vi "K_S30 CalculateCRC16.vi"(7 "msg without CRC":u8[](array[numeric])) -> (0 "CRC16":u16, 1 "CRC Lo":u8, 2 "CRC Hi":u8, 3 "msg and CRC":u8[](array[numeric]))   [LabVIEW 2022 SP3]
panel:
  # "Calculate CRC-16 checksum and append it to the message\nV1.0, b.v."
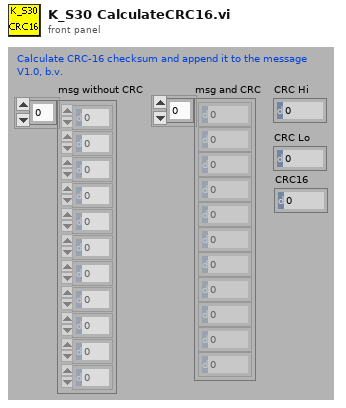
[diagram p1: front panel]
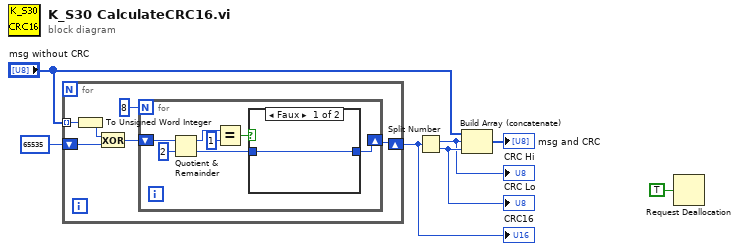
[diagram p0: block diagram]
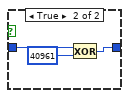
[diagram p2: hidden frame]
diagram:
  n1 = for {
    tunnel: "msg without CRC" -> [w13] mode=indexing
    shift-right: [w9] -> w4
    shift-left: u16 65535 -> [w10]
    n2 = To Unsigned Word Integer(number=w13) -> (unsigned 16bit integer=w8:u16)
    n3 = Exclusive Or(1:w10, 2:w8) -> (0:w11:u16)
    n4 = for {
      N: 8 -> [_]
      shift-right: [w14] -> w9
      shift-left: w11 -> [w20]
      n5 = Quotient & Remainder(x=w20, y=u16 2) -> (x-y*floor(x/y)=w18:u16, floor(x/y)=w15:u16)
      n6 = Equal?(x=w18, y=u16 1) -> (x = y?=w16:bool)
      n7 = case shown="Faux" w16 {
        tunnel: w15 -> [w21 w24]
        tunnel: [w21 w22] -> w14
        frame False {
        }
        frame True {
          n8 = Exclusive Or(1:u16 40961, 2:w24) -> (0:w22:u16)
        }
      }
    }
  }
  "CRC16" <- w4
  n9 = Split Number(x=w4) -> (hi(x)=w2:u8, lo(x)=w3:u8)
  "CRC Hi" <- w2
  "CRC Lo" <- w3
  n10 = Build Array (concatenate)("msg without CRC", w2, w3) -> (→"msg and CRC":u8[])
  n11 = Request Deallocation(TRUE ("flag")) -> ()
